vi "VHist - Fit DBL history to new timestamps.vi"(4 "interpolate (F)":bool, 6 "NaN for absent (F)":bool, 7 "new time stamps":dbl[](array[numeric]) format="%<%H:%M:%S%2u\n%d/%m/%Y>T", 8 "error in":errorcluster, 9 "time condition":cluster{"From":dbl, "To":dbl, "step, sec":dbl} {"step, sec" format="%.2f"; "To" format="%<%H:%M:%S%2u\n%d/%m/%Y>T"; "From" format="%<%H:%M:%S%2u\n%d/%m/%Y>T"}, 10 "history data":dbl[](array[numeric]) format="%.2f", 11 "time stamps":dbl[](array[numeric]) format="%<%H:%M:%S%2u\n%d/%m/%Y>T") -> (0 "error out":errorcluster, 2 "history data out":dbl[](array[numeric]) format="%.2f", 3 "time stamps out":dbl[](array[numeric]) format="%<%H:%M:%S%2u\n%d/%m/%Y>T")   [LabVIEW 2021]
doc: "The VI looks over DBL history and determines history values at the new time stamps specified. New time stamps can be specified either in <b>new time stamps</b> array or <b>time conditions</b> cluster defining initial and final timestamps, and time step. Optionally, VI can interpolate absent values or replace them with NaN.\n\n::: CalcExpress Toolkit :::\nCopyright (c) 2000-2026 Konstantin Shifershteyn. All rights reserved."
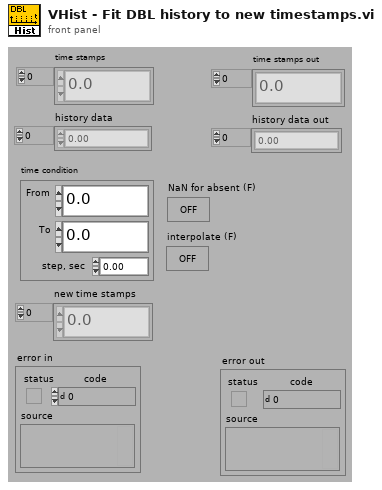
[diagram p1: front panel]
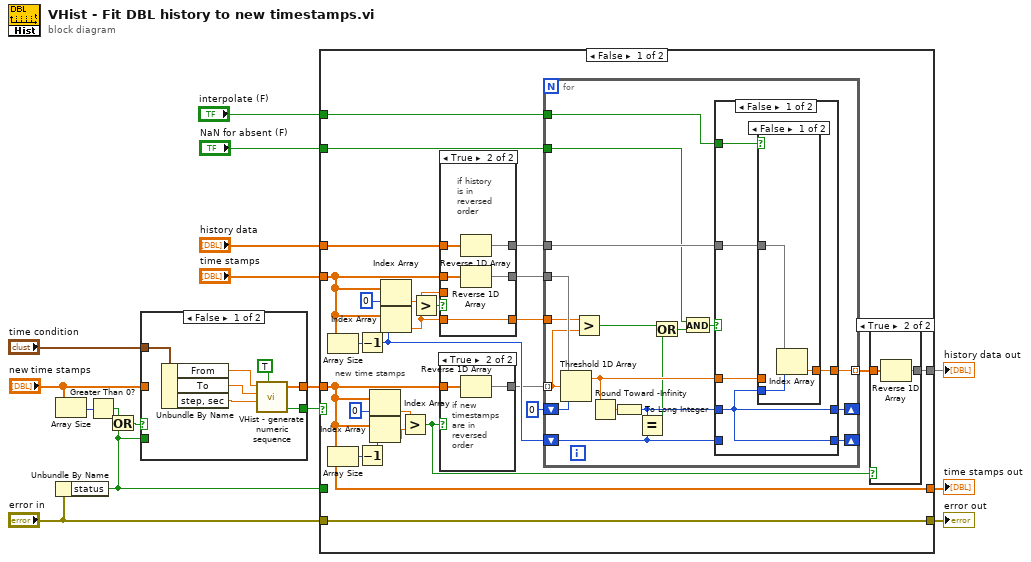
[diagram p0: block diagram]
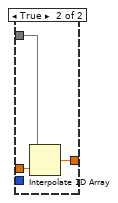
[diagram p6: hidden frame]
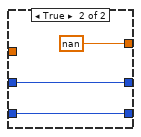
[diagram p7: hidden frame]
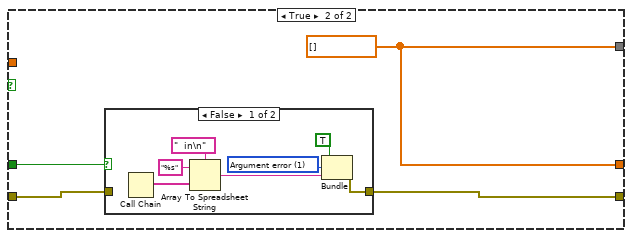
[diagram p8: hidden frame]
diagram:
  n1 = Array Size(array="new time stamps") -> (size(s)=w12:i32)
  n2 = Unbundle By Name("error in") -> ("status"=w3:bool)
  n3 = Greater Than 0?(x=w12) -> (x > 0?=w11:bool)
  n4 = Or(x=w11, y=w3) -> (x .or. y?=w4:bool)
  n5 = case shown="False" w4 {
    tunnel: [w22 w25] -> w8
    tunnel: "new time stamps" -> [_ w25]
    tunnel: "time condition" -> [w23 _]
    tunnel: [w17 w24] -> w7
    tunnel: w3 -> [_ w24]
    frame False {
      n6 = Unbundle By Name(w23) -> ("From"=w19:dbl, "To"=w20:dbl, "step, sec"=w21:dbl)
      n7 = call "VHist - generate numeric sequence.vi"("inclusive (T)"=TRUE, "step"=w21, "final value"=w20, "initial value"=w19) -> ("error"=w17:bool, "array out"=w22:dbl[])  [unwired: 4 in]
    }
    frame True {
    }
  }
  n8 = case shown="False" w7 {
    tunnel: "error in" -> [w50 w99]
    tunnel: w3 -> [_ w100]
    tunnel: [w50 w98] -> w15
    tunnel: [w31 w97] -> w14
    tunnel: [w32 w97] -> w13
    tunnel: w8 -> [w31 _]
    tunnel: "time stamps" -> [w42 _]
    tunnel: "history data" -> [w41 _]
    tunnel: "interpolate (F)" -> [w27 _]
    tunnel: "NaN for absent (F)" -> [w26 _]
    frame False {
      # "new time stamps"
      n9 = Array Size(array=w42) -> (size(s)=w47:i32)
      n10 = Array Size(array=w31) -> (size(s)=w36:i32)
      n11 = Decrement(x=w47) -> (x-1=w44:i32)
      n12 = Decrement(x=w36) -> (x-1=w37:i32)
      n13 = Index Array(array=w31, index=0) -> (element=w39:dbl)
      n14 = Index Array(array=w31, index=w37) -> (element=w40:dbl)
      n15 = Index Array(array=w42, index=0) -> (element=w30:dbl)
      n16 = Index Array(array=w42, index=w44) -> (element=w28:dbl)
      n17 = Greater?(x=w39, y=w40) -> (0:w35:bool)
      n18 = Greater?(x=w30, y=w28) -> (0:w48:bool)
      n19 = case shown="True" w48 {
        tunnel: w42 -> [w59 w64]
        tunnel: [w59 w63] -> w46
        tunnel: w41 -> [w58 w62]
        tunnel: [w58 w61] -> w45
        tunnel: [w57 w60] -> w29
        tunnel: w30 -> [w57 _]
        tunnel: w28 -> [_ w60]
        frame False {
        }
        frame True {
          # "if history\nis in\nreversed\norder"
          n20 = Reverse 1D Array(array=w62) -> (reversed array=w61:dbl[])
          n21 = Reverse 1D Array(array=w64) -> (reversed array=w63:dbl[])
        }
      }
      n22 = case shown="True" w35 {
        tunnel: w31 -> [w54 w56]
        tunnel: [w54 w55] -> w34
        frame False {
        }
        frame True {
          # "if new\ntimestamps\nare in\nreversed\norder"
          n23 = Reverse 1D Array(array=w56) -> (reversed array=w55:dbl[])
        }
      }
      n24 = for {
        tunnel: w45 -> [w82]
        tunnel: w46 -> [w81]
        tunnel: w34 -> [w72] mode=indexing
        tunnel: [w80] -> w33 mode=indexing
        shift-right: [w74] -> _
        shift-left: 0 -> [w78]
        shift-right: [w68] -> _
        shift-left: w44 -> [w67]
        tunnel: w29 -> [w73]
        tunnel: w27 -> [w66]
        tunnel: w26 -> [w65]
        n25 = Threshold 1D Array(1:w78, 2:w72, 3:w81) -> (0:w79:dbl)
        n26 = Greater?(x=w73, y=w72) -> (0:w71:bool)
        n27 = Round Toward -Infinity(1:w79) -> (0:w77:dbl)
        n28 = To Long Integer(number=w77) -> (32bit integer=w75:i32)
        n29 = Equal?(x=w75, y=w67) -> (x = y?=w70:bool)
        n30 = Or(x=w71, y=w70) -> (x .or. y?=w69:bool)
        n31 = And(x=w65, y=w69) -> (x .and. y?=w76:bool)
        n32 = case shown="False" w76 {
          tunnel: w82 -> [w87 _]
          tunnel: [w86 nan ("value")] -> w80
          tunnel: w66 -> [w85 _]
          tunnel: w79 -> [w84 _]
          tunnel: w75 -> [w83 w95]
          tunnel: [w83 w95] -> w74
          tunnel: [w83 w94] -> w68
          tunnel: w67 -> [_ w94]
          frame False {
            n33 = case shown="False" w85 {
              tunnel: w87 -> [w90 w93]
              tunnel: w84 -> [_ w92]
              tunnel: [w89 w91] -> w86
              tunnel: w83 -> [w88 _]
              frame False {
                n34 = Index Array(array=w90, index=w88) -> (element=w89:dbl)
              }
              frame True {
                n35 = Interpolate 1D Array(1:w92, 2:w93) -> (0:w91:dbl)
              }
            }
          }
          frame True {
          }
        }
      }
      n36 = case shown="True" w35 {
        tunnel: w33 -> [w51 w53]
        tunnel: [w51 w52] -> w32
        frame False {
        }
        frame True {
          n37 = Reverse 1D Array(array=w53) -> (reversed array=w52:dbl[])
        }
      }
    }
    frame True {
      w97 = dbl[] []
      n38 = case shown="False" w100 {
        tunnel: [w107 w108] -> w98
        tunnel: w99 -> [_ w108]
        frame False {
          w105 = 1 items=["No error", "Argument error", "Memory is full", "Out of zone", "End of file", "File already open", "Generic file I/O error", "File not found", "File permission error", "Disk is full", "Duplicate path", "Too many files open", "System feature not enabled", "Resource file not found", "Cannot add resource", "Resource not found", "Image not found", "Image memory error", "Pen does not exist", "Config type invalid", "Config token not found", "Config parse error", "Config memory error", "Bad external code format", "Bad external code offset", "External code not present", "Null window", "Destroy window error", "Null menu", "Print aborted", "Bad print record", "Print driver error", "Windows error during printing", "Memory error during printing", "Print dialog error", "Generic print error", "Invalid device refnum", "Device not found", "Device parameter error", "Device unit error", "Cannot open device", "Device call aborted", "Generic error", "Cancelled by user", "Object ID too low", "Object ID too high", "Object not in heap", "Unknown heap", "Unknown object (invalid DefProc)", "Unknown object (DefProc not in table)", "Message out of range", "Invalid (null) method", "Unknown message", "Manager call not supported", "Bad address", "Network operation in progress", "Network operation timed out", "Connection is busy", "Network attribute not supported", "Network error", "Address in use", "System out of memory", "Connection aborted", "Connection refused", "Not connected", "Already connected", "Connection closed", "Initialization error (interapplication manager)", "Bad occurrence", "Wait on unbound occurrence handler", "Occurrence queue overflow", "Datalog type conflict", "Unused", "Unrecognized type (interapplication manager)", "Memory corrupt", "Failed to make temporary DLL", "Old CIN version", "Drag socket not found", "Failed to load drop-object", "Failed to register OLE object", "Failed to release OLE object", "Format specifier type mismatch", "Unknown format specifier", "Too few format specifiers", "Too many format specifiers", "Scan failed", "Newer CIN version", "Error converting to variant", "Runtime menu error", "Password tampered", "Variant attribute not found", "Incompatible variant data type", "Event data is not available", "Event Store is not present", "Occurrence is not found", "Event Queue is not created", "Event info is not available", "Refnum passed is NULL", "Error retrieving Class GUID", "Error retrieving CoClass GUID", "Error retrieving TypeLib GUID.", "Bad built application magic bytes.", "Specific driver is different from the specific driver associated with the Logical Name.", "There is no session opened to the class driver.", "Max Error", "MAX - Error with config objects", "MAX - Error loading configuration", "MAX - Group not supported"]
          n39 = Call Chain() -> (call chain=w104:string[])
          n40 = Array To Spreadsheet String(delimiter (Tab)="  in\n", array=w104, 3:"%s" ("format string")) -> (spreadsheet string=w101:string)
          n41 = Bundle(TRUE, w105, "spreadsheet string"=w101) -> (w107:cluster{bool, i32, "spreadsheet string":string})  [unwired: 1 in]
        }
        frame True {
        }
      }
    }
  }
  "error out" <- w15
  "history data out" <- w13
  "time stamps out" <- w14
